vi "run.vi"(5 "RunGlobalTearDown":bool, 7 "RunGlobalSetup":bool, 8 "error in (no error)":errorcluster, 10 "TestResult in (None: Create New)":refnum<class "TestResult.lvclass">, 11 "TestCase in":refnum<class "TestCase.lvclass">) -> (0 "error out":errorcluster, 2 "TestResult out":refnum<class "TestResult.lvclass">, 3 "TestCase out":refnum<class "TestCase.lvclass">)   [LabVIEW 2013, in "TestCase.lvclass"]
uses:
  TestCase.lvclass
  TestResult/TestResult.lvclass
  TestCase.lvclass/TestCase.ctl
  private/method--Enum.ctl
  JKI Reuse/Is an Error (error cluster)__jki_lib_error_handling -- VI Tester.vi
  Libraries/VITesterUtilities.lvlib
panel:
  # "JKI VI Tester for LabVIEW\nhttp://jkisoft.com/vi-tester\nCopyright (C) 2007-2009, JKI <info@jkisoft.com>\nALL RIGHTS RESERVED"
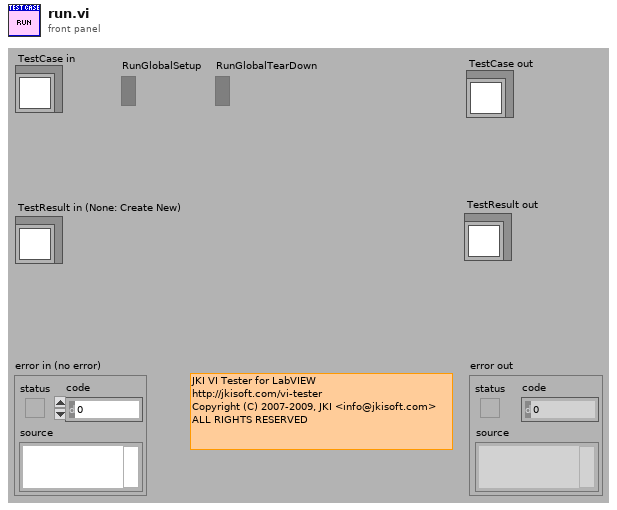
[diagram p1: front panel]
types:
  T1 = typedef "TestCase.lvclass/method--Enum.ctl" = enum16{"setUp", "testMethod", "tearDown"}
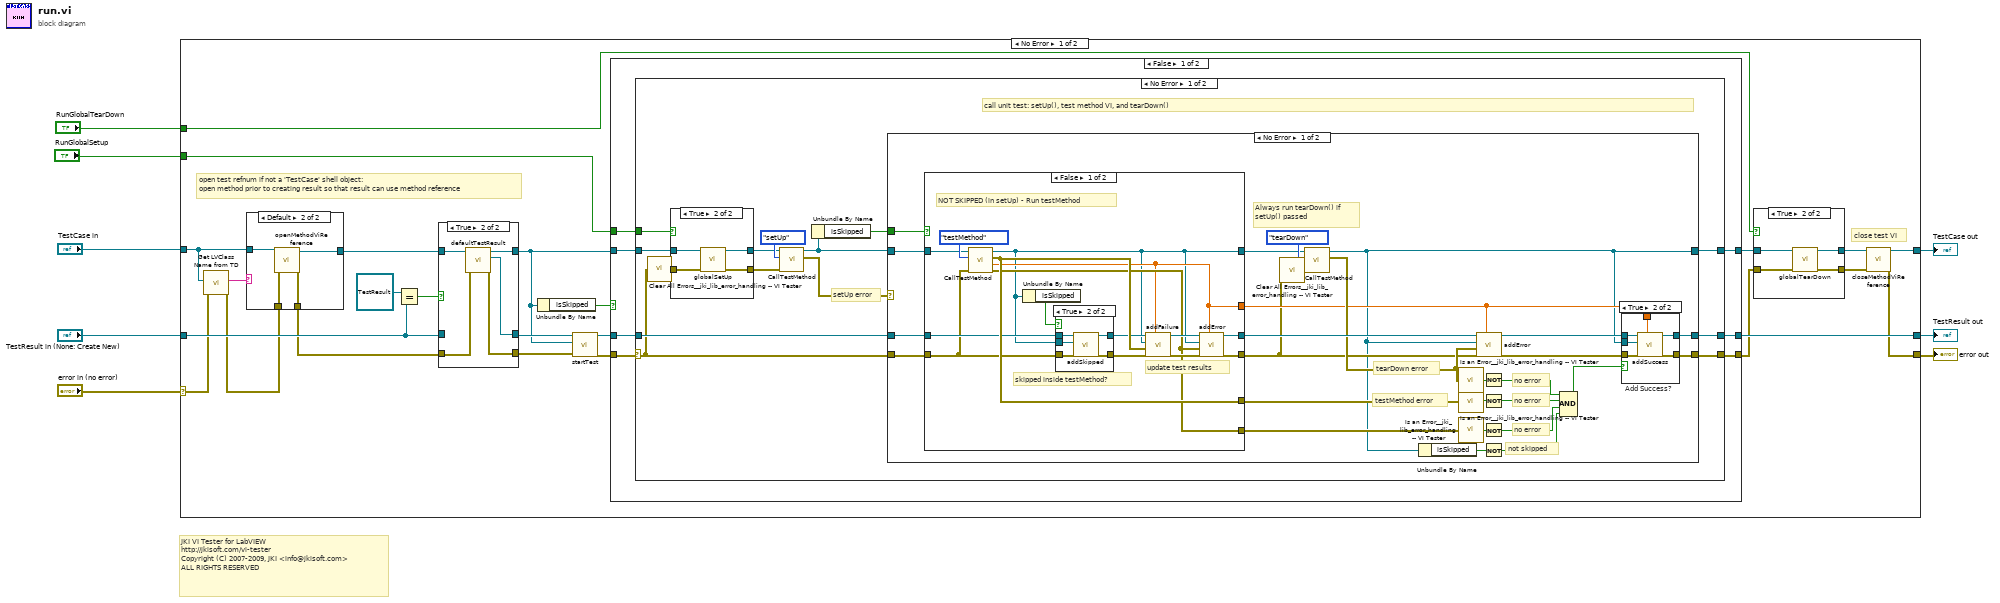
[diagram p0: block diagram]
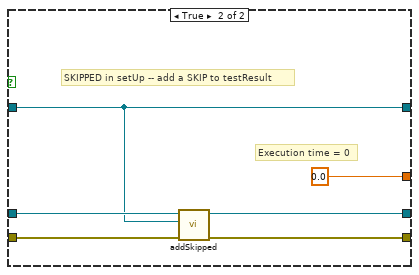
[diagram p6: hidden frame]
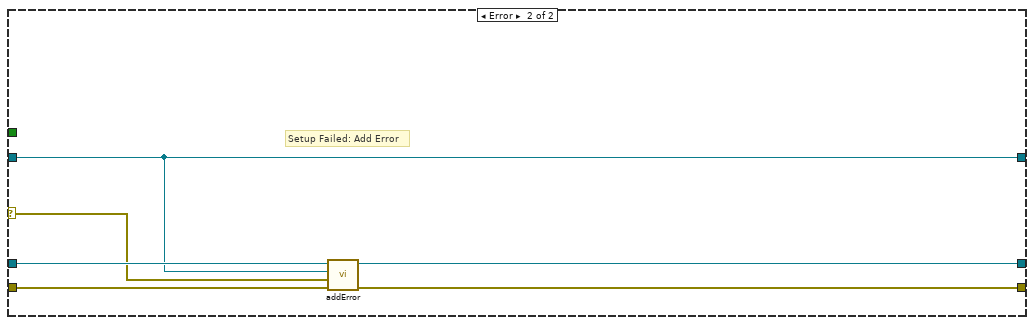
[diagram p8: hidden frame]
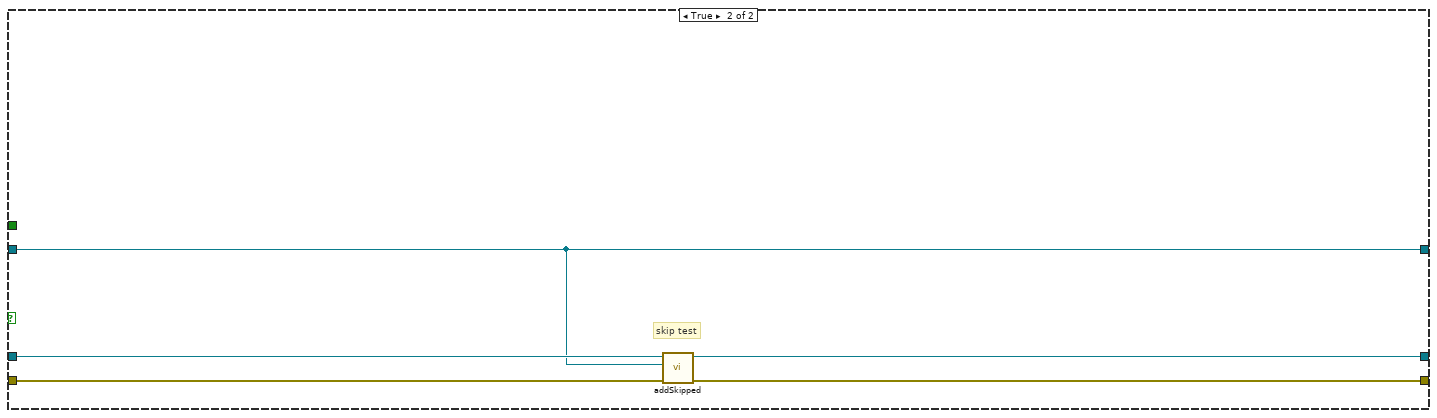
[diagram p10: hidden frame]
diagram:
  # "JKI VI Tester for LabVIEW\nhttp://jkisoft.com/vi-tester\nCopyright (C) 2007-2009, JKI <info@jkisoft.com>\nALL RIGHTS RESERVED"
  n1 = case shown="No Error" "error in (no error)" {
    selector: "error in (no error)" -> [w19 w159]
    tunnel: [w21 w159] -> w7
    tunnel: [w22 w158] -> w5
    tunnel: "TestCase in" -> [w20 w158]
    tunnel: "TestResult in (None: Create New)" -> [w30 w157]
    tunnel: [w29 w157] -> w3
    tunnel: "RunGlobalSetup" -> [w17 _]
    tunnel: "RunGlobalTearDown" -> [w12 _]
    frame No Error {
      # "close test VI"
      # "open test refnum if not a 'TestCase' shell object:\nopen method prior to creating result so that result can use method reference"
      n2 = call "Get LVClass Name from TD.vi"("error in"=w19, "Variant"=w20) -> ("error out"=w18:errorcluster, "LVClass Name"=w25:string)  [unwired: 8 in]
      n3 = case shown="Default" w25 {
        tunnel: w18 -> [w39 w44]
        tunnel: [w40 w43] -> w23
        tunnel: [w39 w42] -> w24
        tunnel: w20 -> [w40 w41]
        frame "TestCase.lvclass" {
        }
        frame Default {
          n4 = call "openMethodViReference.vi"("error in (no error)"=w44, "TestCase in"=w41) -> ("error out"=w42:errorcluster, "TestCase out"=w43:refnum<class "TestCase.lvclass">)  [unwired: 8 in]
        }
      }
      n5 = Equal?(x=refnum<class "TestResult.lvclass"> refnum ("result (None: Create New)"), y=w30) -> (x = y?=w31:bool)
      n6 = case shown="True" w31 {
        tunnel: w23 -> [w151 w156]
        tunnel: [w151 w155] -> w10
        tunnel: [w150 w154] -> w27
        tunnel: w30 -> [w150 _]
        tunnel: w24 -> [w149 w153]
        tunnel: [w149 w152] -> w11
        frame False {
        }
        frame True {
          n7 = call-dynamic "defaultTestResult.vi"("error in (no error)"=w153, "TestCase in"=w156) -> ("error out"=w152:errorcluster, "TestResult"=w154:refnum<class "TestResult.lvclass">, "TestCase out"=w155:refnum<class "TestCase.lvclass">)  [unwired: 7 in]
        }
      }
      n8 = Unbundle By Name(w10) -> ("isSkipped"=w9:bool)
      n9 = call-dynamic "startTest.vi"("error in (no error)"=w11, "test"=w10, "TestResult in"=w27) -> ("error out"=w28:errorcluster, "TestResult in"=w26:refnum<class "TestResult.lvclass">)  [unwired: 7 in]
      n10 = case shown="False" w9 {
        tunnel: w26 -> [w49 w148]
        tunnel: w28 -> [w48 w147]
        tunnel: [w46 w144] -> w16
        tunnel: [w47 w146] -> w14
        tunnel: [w51 w145] -> w29
        tunnel: w10 -> [w50 w144]
        tunnel: w17 -> [w45 _]
        frame False {
          n11 = case shown="No Error" w48 {
            selector: w48 -> [w59 w142]
            tunnel: w50 -> [w56 w143]
            tunnel: [w63 w143] -> w46
            tunnel: w49 -> [w65 w141]
            tunnel: [w64 w142] -> w47
            tunnel: [w62 w141] -> w51
            tunnel: w45 -> [w54 _]
            frame No Error {
              # "setUp error"
              # "call unit test: setUp(), test method VI, and tearDown()"
              n12 = call "Clear All Errors__jki_lib_error_handling -- VI Tester.vi"("error in"=w59) -> ("no error out"=w58:errorcluster)  [unwired: 4 in]
              n13 = case shown="True" w54 {
                tunnel: w58 -> [w66 w70]
                tunnel: [w66 w69] -> w57
                tunnel: w56 -> [w67 w71]
                tunnel: [w67 w68] -> w55
                frame False {
                }
                frame True {
                  n14 = call-dynamic "globalSetUp.vi"("error in (no error)"=w70, "TestCase in"=w71) -> ("error out"=w69:errorcluster, "TestCase out"=w68:refnum<class "TestCase.lvclass">)  [unwired: 8 in]
                }
              }
              n15 = call "CallTestMethod.vi"("error in"=w57, "method"=method--Enum."setUp", "TestCase in"=w55) -> ("Test Method Error"=w60:errorcluster, "TestCase out"=w53:refnum<class "TestCase.lvclass">)  [unwired: 5 in, 2 out]
              n16 = Unbundle By Name(w53) -> ("isSkipped"=w52:bool)
              n17 = case shown="No Error" w60 {
                selector: w60 -> [_ w138]
                tunnel: w65 -> [w81 w140]
                tunnel: w59 -> [w76 w139]
                tunnel: [w92 w136] -> w64
                tunnel: w53 -> [w74 w137]
                tunnel: [w72 w137] -> w63
                tunnel: [w90 w135] -> w62
                tunnel: w52 -> [w75 _]
                frame No Error {
                  # "not skipped"
                  # "no error"
                  # "testMethod error"
                  # "tearDown error"
                  # "no error"
                  # "no error"
                  # "Always run tearDown() if setUp() passed"
                  n18 = case shown="False" w75 {
                    tunnel: [w112 w124] -> w98
                    tunnel: [w110 _] -> w88
                    tunnel: [w108 _] -> w83
                    tunnel: w81 -> [w106 w125]
                    tunnel: [w100 w121] -> w80
                    tunnel: [w104 0.0 ("execution time (sec)")] -> w78
                    tunnel: [w103 w123] -> w77
                    tunnel: w74 -> [w102 w121]
                    tunnel: w76 -> [w101 w126]
                    frame False {
                      # "skipped inside testMethod?"
                      # "NOT SKIPPED (in setUp) - Run testMethod"
                      # "update test results"
                      n19 = call "CallTestMethod.vi"("error in"=w101, "method"=method--Enum."testMethod", "TestCase in"=w102) -> ("error out"=w108:errorcluster, "execution time (sec)"=w104:dbl, "Test Method Error"=w110:errorcluster, "TestCase out"=w100:refnum<class "TestCase.lvclass">)  [unwired: 5 in]
                      n20 = Unbundle By Name(w100) -> ("isSkipped"=w99:bool)
                      n21 = case shown="True" w99 {
                        tunnel: w101 -> [w114 w120]
                        tunnel: [w114 w119] -> w107
                        tunnel: w106 -> [w115 w118]
                        tunnel: [w115 w117] -> w105
                        tunnel: w100 -> [_ w116]
                        frame False {
                        }
                        frame True {
                          n22 = call-dynamic "addSkipped.vi"("error in (no error)"=w120, "test"=w116, "TestResult in"=w118) -> ("error out"=w119:errorcluster, "TestResult out"=w117:refnum<class "TestResult.lvclass">)  [unwired: 7 in]
                        }
                      }
                      n23 = call-dynamic "addFailure.vi"("execution time (sec)"=w104, "error in (no error)"=w107, "test error"=w110, "test"=w100, "TestResult in"=w105) -> ("error out"=w111:errorcluster, "TestResult out"=w113:refnum<class "TestResult.lvclass">)  [unwired: 5 in]
                      n24 = call-dynamic "addError.vi"("execution time (sec)"=w104, "error in (no error)"=w111, "test error"=w108, "test"=w100, "TestResult in"=w113) -> ("error out"=w103:errorcluster, "TestResult out"=w112:refnum<class "TestResult.lvclass">)  [unwired: 5 in]
                    }
                    frame True {
                      # "Execution time = 0"
                      # "SKIPPED in setUp -- add a SKIP to testResult"
                      n25 = call-dynamic "addSkipped.vi"("error in (no error)"=w126, "test"=w121, "TestResult in"=w125) -> ("error out"=w123:errorcluster, "TestResult out"=w124:refnum<class "TestResult.lvclass">)  [unwired: 7 in]
                    }
                  }
                  n26 = call "Clear All Errors__jki_lib_error_handling -- VI Tester.vi"("error in"=w77) -> ("no error out"=w87:errorcluster)  [unwired: 4 in]
                  n27 = call "CallTestMethod.vi"("error in"=w87, "method"=method--Enum."tearDown", "TestCase in"=w80) -> ("Test Method Error"=w85:errorcluster, "TestCase out"=w72:refnum<class "TestCase.lvclass">)  [unwired: 5 in, 2 out]
                  n28 = Unbundle By Name(w72) -> ("isSkipped"=w73:bool)
                  n29 = call-poly "Is an Error__jki_lib_error_handling -- VI Tester.vi"("error in"=w85) -> ("error?"=w97:bool)  [unwired: 8 in]
                  n30 = call-poly "Is an Error__jki_lib_error_handling -- VI Tester.vi"("error in"=w88) -> ("error?"=w89:bool)  [unwired: 8 in]
                  n31 = call-poly "Is an Error__jki_lib_error_handling -- VI Tester.vi"("error in"=w83) -> ("error?"=w84:bool)  [unwired: 8 in]
                  n32 = call-dynamic "addError.vi"("execution time (sec)"=w78, "error in (no error)"=w77, "test error"=w85, "test"=w72, "TestResult in"=w98) -> ("error out"=w93:errorcluster, "TestResult out"=w94:refnum<class "TestResult.lvclass">)  [unwired: 5 in]
                  n33 = Not(x=w97) -> (.not. x?=w96:bool)
                  n34 = Not(x=w89) -> (.not. x?=w95:bool)
                  n35 = Not(x=w84) -> (.not. x?=w82:bool)
                  n36 = Not(x=w73) -> (.not. x?=w79:bool)
                  n37 = Compound Arithmetic op=AND(w96, w95, w82, w79) -> (w91:bool)
                  n38 = case "Add Success?" shown="True" w91 {
                    tunnel: w94 -> [w128 w134]
                    tunnel: w93 -> [w127 w133]
                    tunnel: [w127 w132] -> w92
                    tunnel: [w128 w131] -> w90
                    tunnel: w72 -> [_ w130]
                    tunnel: w78 -> [_ w129]
                    frame False {
                    }
                    frame True {
                      n39 = call-dynamic "addSuccess.vi"("execution time (sec)"=w129, "error in (no error)"=w133, "test"=w130, "TestResult in"=w134) -> ("error out"=w132:errorcluster, "TestResult in"=w131:refnum<class "TestResult.lvclass">)  [unwired: 6 in]
                    }
                  }
                }
                frame Error {
                  # "Setup Failed: Add Error"
                  n40 = call-dynamic "addError.vi"("error in (no error)"=w139, "test error"=w138, "test"=w137, "TestResult in"=w140) -> ("error out"=w136:errorcluster, "TestResult out"=w135:refnum<class "TestResult.lvclass">)  [unwired: 6 in]
                }
              }
            }
            frame Error {
            }
          }
        }
        frame True {
          # "skip test"
          n41 = call-dynamic "addSkipped.vi"("error in (no error)"=w147, "test"=w144, "TestResult in"=w148) -> ("error out"=w146:errorcluster, "TestResult out"=w145:refnum<class "TestResult.lvclass">)  [unwired: 7 in]
        }
      }
      n42 = case shown="True" w12 {
        tunnel: w14 -> [w33 w37]
        tunnel: [w33 w35] -> w13
        tunnel: w16 -> [w34 w38]
        tunnel: [w34 w36] -> w15
        frame False {
        }
        frame True {
          n43 = call-dynamic "globalTearDown.vi"("error in (no error)"=w37, "TestCase in"=w38) -> ("error out"=w35:errorcluster, "TestCase out"=w36:refnum<class "TestCase.lvclass">)  [unwired: 8 in]
        }
      }
      n44 = call "closeMethodViReference.vi"("error in (no error)"=w13, "TestCase in"=w15) -> ("error out"=w21:errorcluster, "TestCase in"=w22:refnum<class "TestCase.lvclass">)  [unwired: 8 in]
    }
    frame Error {
    }
  }
  "error out" <- w7
  "TestCase out" <- w5
  "TestResult out" <- w3
